vi "AlliGator Parameter Map Event Registration Refnums.vi"(8 "error in (no error)":errorcluster) -> (0 "error out":errorcluster, 2 "Parameter Map Display Event":refnum<event-registration>, 3 "Parameter Map Display Range Event":refnum<event-registration>)   [LabVIEW 2021, in "AlliGator Parameter Map.lvlib"]
uses:
  AlliGator Parameter Map.lvlib
panel:
  # "see the License on the block diagram (Ctrl+E or Window:Show Block Diagram)"
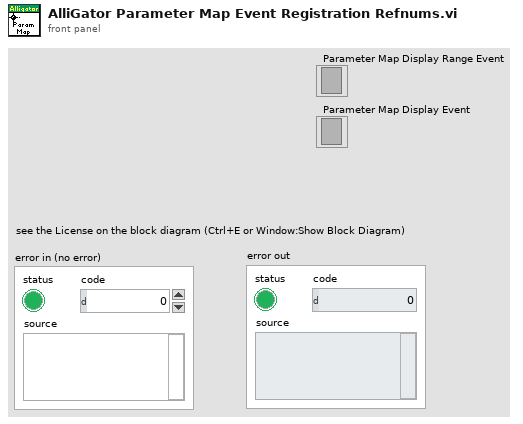
[diagram p1: front panel]
types:
  T1 = typedef "AlliGator Parameter Map.lvlib/AlliGator Parameter Map Control Refnums.ctl" = cluster{"Parameter Map Color Scale":refnum<vi>, "Map Parameter":refnum<vi>, "Max Parameter":refnum<vi>, "Min Parameter":refnum<vi>, "Parameter Map Display":refnum<vi>, "Parameter Map Display Range":refnum<vi>, "Parameter Map Set":refnum<vi>, "Parameter Map X":refnum<vi>, "Parameter Map Y":refnum<vi>, "Parameter Map Value":refnum<vi>}
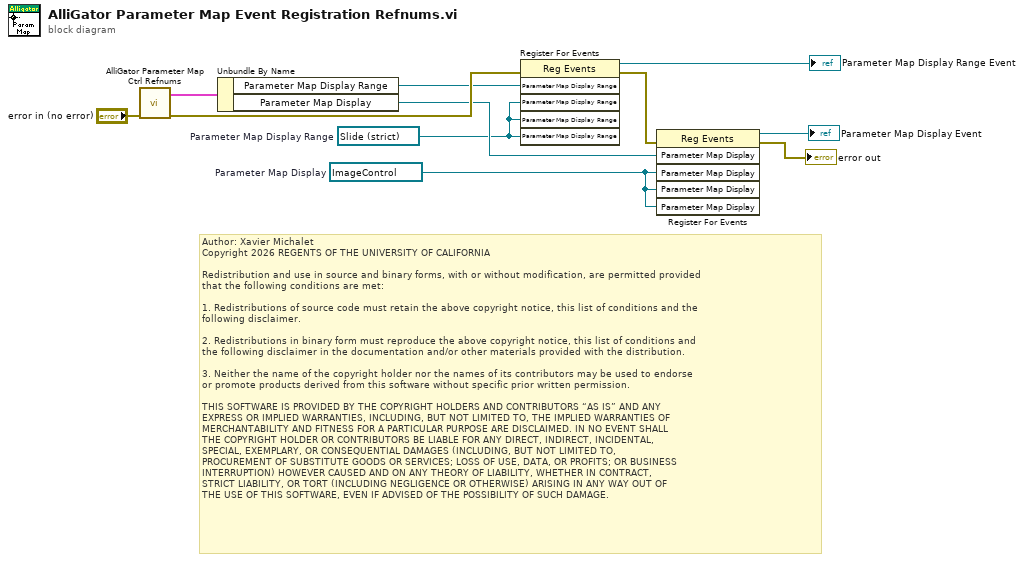
[diagram p0: block diagram]
diagram:
  w2 = refnum<vi> refnum  # Parameter Map Display
  w6 = refnum<vi> refnum  # Parameter Map Display Range
  # "Author: Xavier Michalet\nCopyright 2026 REGENTS OF THE UNIVERSITY OF CALIFORNIA\n\nRedistribution and use in source and binary forms, with or without modification, are permitted provided\nthat the following conditions are met:\n\n1. Redistributions of source code must retain the above copyright notice, this list of conditions and the\nfollowing disclaimer.\n\n2. Redistributions in binary form must reproduce the above copyright notice, this list of conditions and\nthe following disclaimer in the documentation and/or other materials provided with the distribution.\n\n3. Neither the name of the copyright holder nor the names of its contributors may be used to endorse \nor promote products derived from this software without specific prior written permission.\n\nTHIS SOFTWARE IS PROVIDED BY THE COPYRIGHT HOLDERS AND CONTRIBUTORS “AS IS” AND ANY \nEXPRESS OR IMPLIED WARRANTIES, INCLUDING, BUT NOT LIMITED TO, THE IMPLIED WARRANTIES OF\nMERCHANTABILITY AND FITNESS FOR A PARTICULAR PURPOSE ARE DISCLAIMED. IN NO EVENT SHALL\nTHE COPYRIGHT HOLDER OR CONTRIBUTORS BE LIABLE FOR ANY DIRECT, INDIRECT, INCIDENTAL, \nSPECIAL, EXEMPLARY, OR CONSEQUENTIAL DAMAGES (INCLUDING, BUT NOT LIMITED TO, \nPROCUREMENT OF SUBSTITUTE GOODS OR SERVICES; LOSS OF USE, DATA, OR PROFITS; OR BUSINESS\nINTERRUPTION) HOWEVER CAUSED AND ON ANY THEORY OF LIABILITY, WHETHER IN CONTRACT, \nSTRICT LIABILITY, OR TORT (INCLUDING NEGLIGENCE OR OTHERWISE) ARISING IN ANY WAY OUT OF\nTHE USE OF THIS SOFTWARE, EVEN IF ADVISED OF THE POSSIBILITY OF SUCH DAMAGE."
  n1 = call "AlliGator Parameter Map Ctrl Refnums.vi"("error in (no error)"="error in (no error)") -> ("error out"=w11:errorcluster, "Parameter Map Ctrl Refums"=w9:T1)  [unwired: 9 in]
  n2 = Unbundle By Name(w9) -> ("Parameter Map Display Range"=w7:refnum<vi>, "Parameter Map Display"=w8:refnum<vi>)
  n3 = register-events(error in=w11, w7, w6, w6, w6) -> (reference out=→"Parameter Map Display Range Event":refnum<event-registration>, error out=w4:errorcluster)  [unwired: 1 in]
  n4 = register-events(error in=w4, w8, w2, w2, w2) -> (reference out=→"Parameter Map Display Event":refnum<event-registration>, error out=→"error out":errorcluster)  [unwired: 1 in]
